vi "FlatToRichcif_can_writer_nixnet_XnetDevices.vi"(5 "OutputClusterType":T1, 11 "InputCluster":T3) -> (3 "OutputCluster":T1)   [LabVIEW 2021, in "CanWriterNixnet_client.lvlib"]
uses:
  CanWriterNixnet_client.lvlib
  cif_can_writer_nixnet_XnetDevices_Flat.ctl
  cif_can_writer_nixnet_XnetDevice_Flat.ctl
  cif_can_writer_nixnet_XnetDevices.ctl
  cif_can_writer_nixnet_XnetDevice.ctl
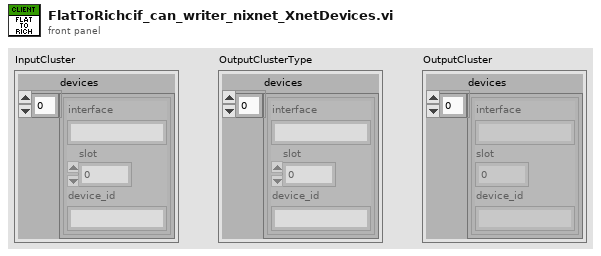
[diagram p1: front panel]
types:
  T1 = typedef "CanWriterNixnet_client.lvlib/cif_can_writer_nixnet_XnetDevices.ctl" = cluster{"devices":T2[]}
  T2 = typedef "CanWriterNixnet_client.lvlib/cif_can_writer_nixnet_XnetDevice.ctl" = cluster{"interface":string, "slot":u32, "device_id":string}
  T3 = typedef "CanWriterNixnet_client.lvlib/cif_can_writer_nixnet_XnetDevices_Flat.ctl" = cluster{"devices":T4[]}
  T4 = typedef "CanWriterNixnet_client.lvlib/cif_can_writer_nixnet_XnetDevice_Flat.ctl" = cluster{"interface":string, "slot":u32, "device_id":string}
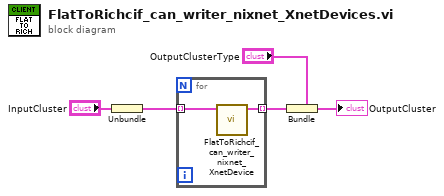
[diagram p0: block diagram]
diagram:
  n1 = Unbundle "Unbundle"("InputCluster") -> ("devices"=w2:T4[])
  n2 = for {
    tunnel: w2 -> [w7] mode=indexing
    tunnel: [w6] -> w1 mode=indexing
    n3 = call "FlatToRichcif_can_writer_nixnet_XnetDevice.vi"("InputCluster"=w7) -> ("OutputCluster"=w6:T2)  [unwired: 10 in]
  }
  n4 = Bundle "Bundle"(cluster="OutputClusterType", "devices"=w1) -> (→"OutputCluster":T1)
